vi "2D w X&Y Macro.vi"(0 "2D wave":string, 1 "minimum":dbl, 2 "maximum":dbl, 5 "X wave":string, 7 "Y wave":string, 9 "X,Y,Z Labels":string[](array[string])=["current (nA)", "field (oe)", "dV/dI (Ohm)"], 11 "error in (no error)":errorcluster, 12 "Kill X&Y waves? [T]":bool=TRUE) -> (4 "ITX Commands out":refnum<class "ITX Commands.lvclass">, 6 "result string":string, 15 "error out":errorcluster)   [LabVIEW 2019, in "ITX Commands.lvclass"]
uses:
  ITX Commands.lvclass
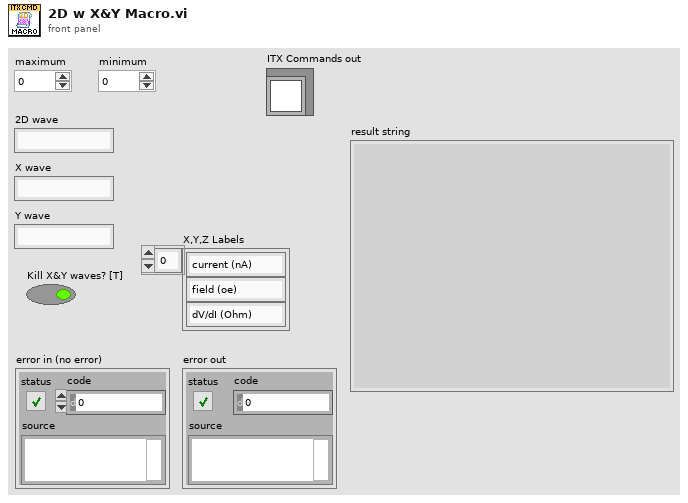
[diagram p1: front panel]
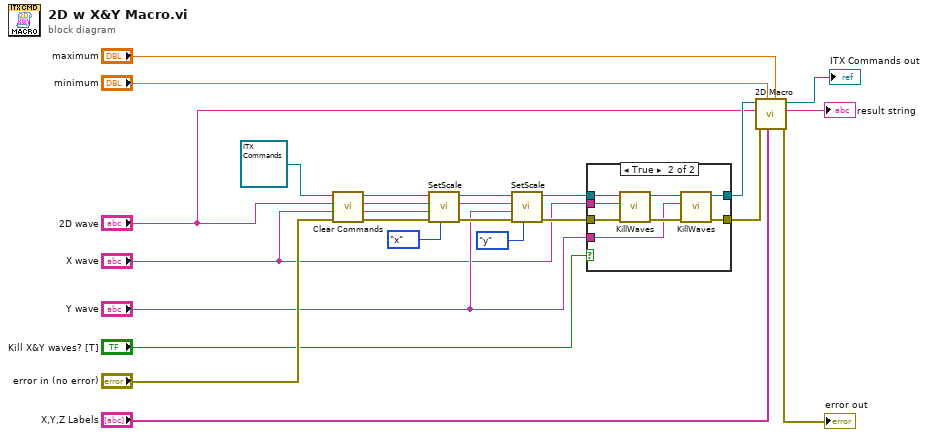
[diagram p0: block diagram]
diagram:
  n1 = call "Clear Commands.vi"("error in (no error)"="error in (no error)", "ITX Commands in"=refnum<class "ITX Commands.lvclass"> refnum) -> ("error out"=w11:errorcluster, "ITX Commands out"=w14:refnum<class "ITX Commands.lvclass">)  [unwired: 8 in]
  n2 = call "SetScale.vi"("Axis"=enum16{"x", "y", "z"}."x", "error in (no error)"=w11, "wavename (Axis)"="X wave", "wavename (Image)"="2D wave", "ITX Commands in"=w14) -> ("error out"=w16:errorcluster, "ITX Commands out"=w15:refnum<class "ITX Commands.lvclass">)  [unwired: 5 in]
  n3 = call "SetScale.vi"("Axis"=enum16{"x", "y", "z"}."y", "error in (no error)"=w16, "wavename (Axis)"="Y wave", "wavename (Image)"="2D wave", "ITX Commands in"=w15) -> ("error out"=w7:errorcluster, "ITX Commands out"=w13:refnum<class "ITX Commands.lvclass">)  [unwired: 5 in]
  n4 = case shown="True" "Kill X&Y waves? [T]" {
    tunnel: w13 -> [w24 w32]
    tunnel: [w24 w29] -> w10
    tunnel: [w23 w28] -> w9
    tunnel: "X wave" -> [_ w27]
    tunnel: w7 -> [w23 w26]
    tunnel: "Y wave" -> [_ w25]
    frame False {
    }
    frame True {
      n5 = call "KillWaves.vi"("error in (no error)"=w26, "wavename"=w27, "ITX Commands in"=w32) -> ("error out"=w30:errorcluster, "ITX Commands out"=w31:refnum<class "ITX Commands.lvclass">)  [unwired: 7 in]
      n6 = call "KillWaves.vi"("error in (no error)"=w30, "wavename"=w25, "ITX Commands in"=w31) -> ("error out"=w28:errorcluster, "ITX Commands out"=w29:refnum<class "ITX Commands.lvclass">)  [unwired: 7 in]
    }
  }
  n7 = call "2D Macro.vi"("maximum"="maximum", "X,Y,Z Labels"="X,Y,Z Labels", "minimum"="minimum", "error in (no error)"=w9, "2D wavename"="2D wave", "ITX Commands in"=w10) -> ("error out"=→"error out":errorcluster, "Commands"=→"result string":string, "ITX Commands out"=→"ITX Commands out":refnum<class "ITX Commands.lvclass">)  [unwired: 3 in]
